vi "Dialog Box.vi"(8 "error in (no error)":errorcluster, 11 "Msg_Error in":refnum<class "Msg_Error.lvclass">) -> (0 "error out":errorcluster, 1 "timed out?":bool, 2 "Selection":string, 3 "Msg_Error out":refnum<class "Msg_Error.lvclass">)   [LabVIEW 2012, in "Msg_Error.lvlib" / "Msg_Error.lvclass"]
doc: "This VI contains the code for the dialog box.\nOverride this VI to provide more functionality or to create your own application-specific dialog box."
uses:
  Msg_Error.lvclass
  Msg_Error.lvclass/Msg_Error.ctl
  <vilib>/Utility/error.llb/DialogType.ctl
  Fading/_Fade In(I32).vi
panel:
  out "String":string
  out "Error Code":string
  in  "Show details":bool
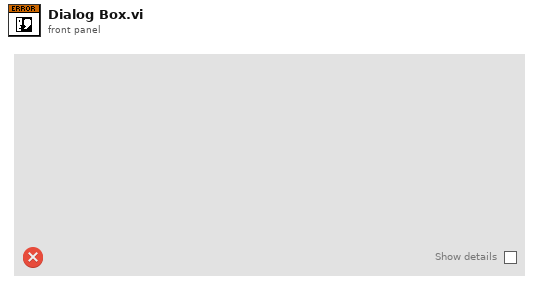
[diagram p1: front panel]
types:
  T1 = typedef "DialogType.ctl" = u16
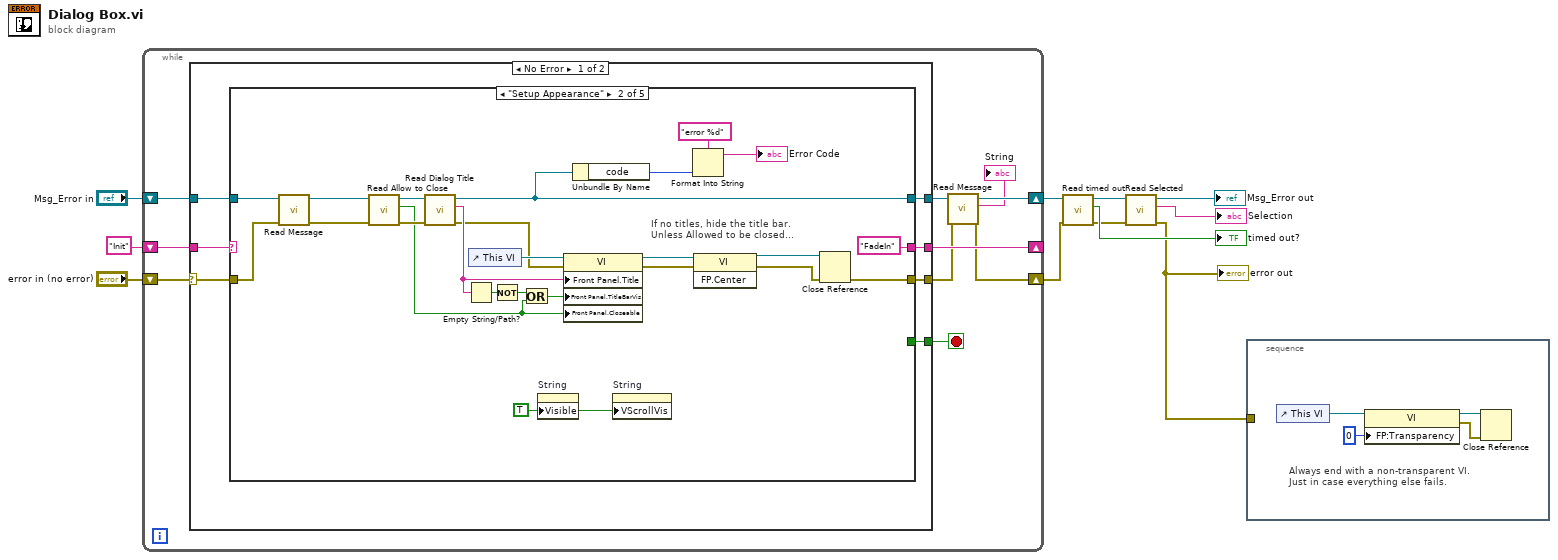
[diagram p0: block diagram]
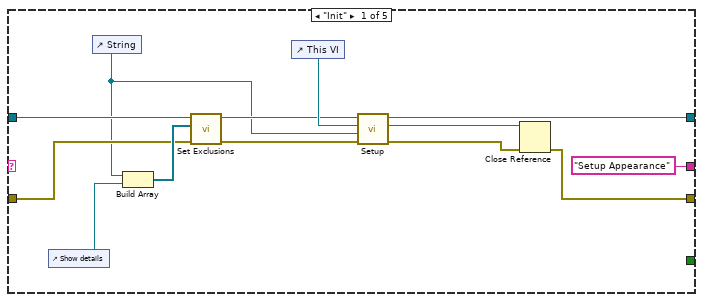
[diagram p2: hidden frame]
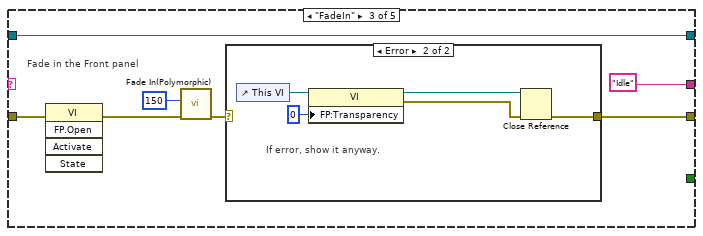
[diagram p3: hidden frame]
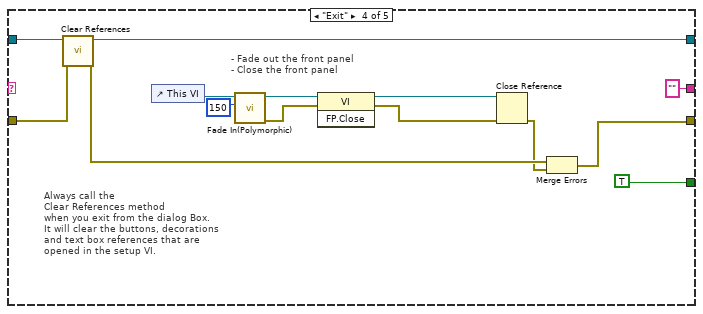
[diagram p5: hidden frame]
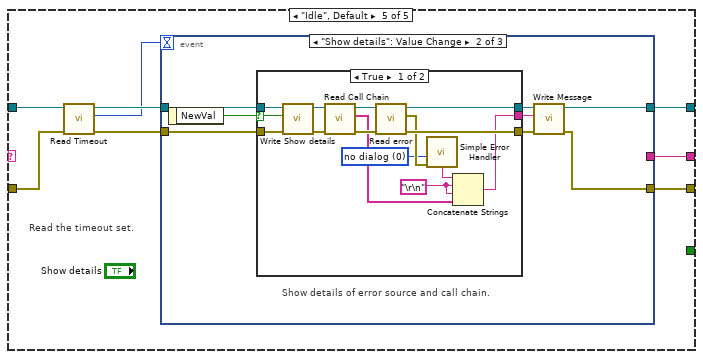
[diagram p6: hidden frame]
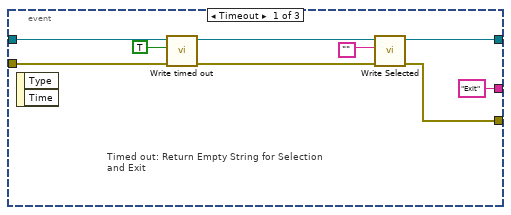
[diagram p7: hidden frame]
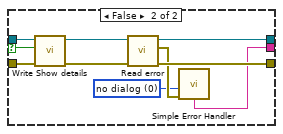
[diagram p8: hidden frame]
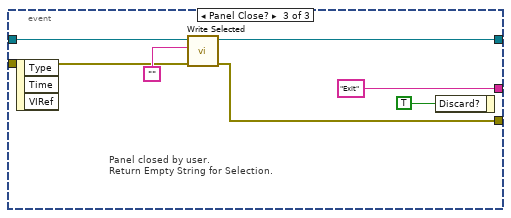
[diagram p9: hidden frame]
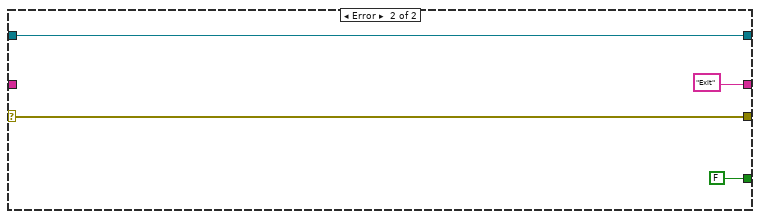
[diagram p10: hidden frame]
diagram:
  n1 = while {
    shift-right: [w19] -> _
    shift-left: "Init" -> [w20]
    shift-right: [w16] -> w5
    shift-left: "Msg_Error in" -> [w21]
    shift-right: [w13] -> w4
    shift-left: "error in (no error)" -> [w17]
    stop <- w18 stop-if-true
    n2 = case shown="No Error" w17 {
      selector: w17 -> [w22 w152]
      tunnel: [w28 w153] -> w15
      tunnel: w21 -> [w27 w153]
      tunnel: [w26 w152] -> w12
      tunnel: w20 -> [w25 _]
      tunnel: [w24 "Exit"] -> w19
      tunnel: [w23 FALSE] -> w18
      frame No Error {
        n3 = case shown="\"Setup Appearance\"" w25 {
          tunnel: [w39 w46 w72 w87 w100] -> w28
          tunnel: w27 -> [w34 w50 w72 w88 w97]
          tunnel: [w40 w57 w68 w86 w99] -> w26
          tunnel: w22 -> [w32 w48 w67 w79 w94]
          tunnel: ["Setup Appearance" "FadeIn" "Idle" "" w98] -> w24
          tunnel: [_ _ _ TRUE _] -> w23
          frame "Init" {
            n4 = control-ref of="Show details"() -> (w29:refnum<vi>)
            n5 = control-ref of="String"() -> (w30:refnum<vi>)
            n6 = Build Array(w30, w29) -> (w35:refnum<vi>[])
            n7 = call-dynamic "Set Exclusions.vi"("error in (no error)"=w32, "Exclusions"=w35, "Dialog in"=w34) -> ("error out"=w31:errorcluster, "Dialog out"=w33:refnum<class "Msg_Error.lvclass">)  [unwired: 7 out]
            n8 = control-ref of="This VI"() -> (w37:refnum<vi>)
            n9 = call-dynamic "Setup.vi"("error in (no error)"=w31, "Str Refnum"=w30, "VI Reference"=w37, "Msg_Error in"=w33) -> ("error out"=w36:errorcluster, "VI reference (dup)"=w38:refnum<vi>, "Msg_Error out"=w39:refnum<class "Msg_Error.lvclass">)  [unwired: 5 out]
            n10 = Close Reference(reference=w38, error in (no error)=w36) -> (error out=w40:errorcluster)
          }
          frame "Setup Appearance" {
            w42 = TRUE ("Visible")
            # "If no titles, hide the title bar.\nUnless Allowed to be closed..."
            n11 = call-dynamic "Read Message.vi"("error in (no error)"=w48, "Dialog in"=w50) -> ("error out"=w47:errorcluster, "Dialog out"=w49:refnum<class "Msg_Error.lvclass">)  [unwired: 7 in, 1 out]
            n12 = call-dynamic "Read Allow to Close.vi"("error in (no error)"=w47, "Dialog.lvclass in"=w49) -> ("error out"=w54:errorcluster, "Allow to close?"=w51:bool, "Dialog.lvclass out"=w55:refnum<class "Msg_Error.lvclass">)  [unwired: 7 out]
            n13 = call-dynamic "Read Dialog Title.vi"("error in (no error)"=w54, "Dialog in"=w55) -> ("error out"=w56:errorcluster, "Dialog Title"=w60:string, "Dialog out"=w46:refnum<class "Msg_Error.lvclass">)  [unwired: 7 out]
            n14 = Empty String/Path?(string/path=w60) -> (empty?=w63:bool)
            n15 = control-ref of="This VI"() -> (w64:refnum<vi>)
            n16 = Not(x=w63) -> (.not. x?=w53:bool)
            n17 = Or(x=w53, y=w51) -> (x .or. y?=w52:bool)
            n18 = property on="String" class="Str"("Visible"=w42) -> ()  [unwired: 2 in, 2 out]
            n19 = property class="VI"(reference=w64, error in=w56, "Front Panel.Title"=w60, "Front Panel.TitleBarVis"=w52, "Front Panel.Closeable"=w51) -> (reference out=w62:refnum<vi>, error out=w61:errorcluster)
            n20 = Unbundle By Name(w46) -> ("code"=w45:i32)
            n21 = property on="String" class="Str"("VScrollVis"=w42) -> ()  [unwired: 2 in, 2 out]
            n22 = Format Into String(format string="error %d", w45) -> (resulting string=→"Error Code":string)  [unwired: 2 in, 1 out]
            n23 = invoke class="VI" method="FP.Center"(reference=w62, error in=w61) -> (reference out=w59:refnum<vi>, error out=w58:errorcluster)  [unwired: 1 in, 1 out]
            n24 = Close Reference(reference=w59, error in (no error)=w58) -> (error out=w57:errorcluster)
          }
          frame "FadeIn" {
            # "Fade in the Front panel"
            n25 = invoke class="VI" method="FP.Open"(error in=w67) -> (error out=w66:errorcluster)  [unwired: 4 in, 4 out]
            n26 = call-poly "Fade In(Polymorphic).vi"("error in"=w66, "Fade time (ms)"=150) -> ("error out"=w69:errorcluster)  [unwired: 2 in, 7 out]
            n27 = case shown="Error" w69 {
              selector: w69 -> [w73 _]
              tunnel: [w73 w74] -> w68
              frame No Error {
              }
              frame Error {
                # "If error, show it anyway."
                n28 = control-ref of="This VI"() -> (w76:refnum<vi>)
                n29 = property class="VI"(reference=w76, "FP:Transparency"=u8 0 ("Front Panel Window:Transparency")) -> (reference out=w77:refnum<vi>, error out=w78:errorcluster)  [unwired: 1 in]
                n30 = Close Reference(reference=w77, error in (no error)=w78) -> (error out=w74:errorcluster)
              }
            }
          }
          frame "Exit" {
            # "Always call the\nClear References method\nwhen you exit from the dialog Box.\nIt will clear the buttons, decorations\nand text box references that are \nopened in the setup VI."
            # "- Fade out the front panel\n- Close the front panel"
            n31 = call-dynamic "Clear References.vi"("error in (no error)"=w79, "Dialog in"=w88) -> ("error out"=w81:errorcluster, "Dialog out"=w87:refnum<class "Msg_Error.lvclass">)  [unwired: 8 out]
            n32 = control-ref of="This VI"() -> (w89:refnum<vi>)
            n33 = call-poly "Fade In(Polymorphic).vi"("Fade time (ms)"=150, "VI Reference (calling VI)"=w89) -> ("error out"=w85:errorcluster, "dup VI Reference"=w84:refnum<vi>)  [unwired: 2 in, 6 out]
            n34 = invoke class="VI" method="FP.Close"(reference=w84, error in=w85) -> (reference out=w82:refnum<vi>, error out=w83:errorcluster)  [unwired: 1 in, 1 out]
            n35 = Close Reference(reference=w82, error in (no error)=w83) -> (error out=w80:errorcluster)
            n36 = Merge Errors(w81, w80) -> (w86:errorcluster)
          }
          frame "Idle", Default {
            # "Read the timeout set."
            n37 = call-dynamic "Read Timeout.vi"("error in (no error)"=w94, "Dialog.lvclass in"=w97) -> ("error out"=w93:errorcluster, "Timeout"=w95:i32, "Dialog.lvclass out"=w96:refnum<class "Msg_Error.lvclass">)  [unwired: 7 out]
            n38 = event shown="[1] \"Show details\": Value Change" {
              selector: _ -> [_ _ _]
              dyn-events: _ -> [_ _ _]
              timeout: w95 -> [_ _ _]
              tunnel: [w102 w115 w145] -> w100
              tunnel: w96 -> [w108 w112 w146]
              tunnel: [w103 w116 w143] -> w99
              tunnel: w93 -> [w106 w111 w144]
              tunnel: ["Exit" _ "Exit"] -> w98
              event Timeout {
                # "Timed out: Return Empty String for Selection\nand Exit"
                n39 = event-data() -> ()  [unwired: 3 out]
                n40 = call-dynamic "Write timed out.vi"("error in (no error)"=w106, "timed out?"=TRUE, "Dialog.lvclass in"=w108) -> ("error out"=w104:errorcluster, "Dialog.lvclass out"=w105:refnum<class "Msg_Error.lvclass">)  [unwired: 7 out]
                n41 = call-dynamic "Write Selected.vi"("error in (no error)"=w104, "Selected"="", "Dialog.lvclass in"=w105) -> ("error out"=w103:errorcluster, "Dialog.lvclass out"=w102:refnum<class "Msg_Error.lvclass">)  [unwired: 7 out]
              }
              event "Show details": Value Change {
                # "Show details of error source and call chain."
                n42 = event-data() -> ("NewVal"=w110:bool)  [unwired: 1 out]
                n43 = case shown="True" w110 {
                  selector: w110 -> [w118 w136]
                  tunnel: [w130 w142] -> w117
                  tunnel: [w129 w133] -> w114
                  tunnel: [w128 w141] -> w113
                  tunnel: w112 -> [w120 w138]
                  tunnel: w111 -> [w119 w137]
                  frame True {
                    w122 = "\r\n"
                    w121 = T1 0 items=["no dialog", "OK message", "continue or stop message", "OK message + warnings", "continue/stop + warnings"] ("type of dialog (OK msg:1)")
                    n44 = call-dynamic "Write Show details.vi"("error in (no error)"=w119, "Show details"=w118, "Msg_Error.lvclass in"=w120) -> ("error out"=w132:errorcluster, "Msg_Error.lvclass out"=w131:refnum<class "Msg_Error.lvclass">)  [unwired: 7 out]
                    n45 = call-dynamic "Read Call Chain.vi"("error in (no error)"=w132, "Msg_Error.lvclass in"=w131) -> ("error out"=w127:errorcluster, "Call Chain"=w126:string[], "Msg_Error.lvclass out"=w125:refnum<class "Msg_Error.lvclass">)  [unwired: 7 out]
                    n46 = call-dynamic "Read error.vi"("error in (no error)"=w127, "Msg_Error.lvclass in"=w125) -> ("error out"=w130:errorcluster, "error"=w124:errorcluster, "Msg_Error.lvclass out"=w128:refnum<class "Msg_Error.lvclass">)  [unwired: 7 out]
                    n47 = call <vilib>:"Simple Error Handler.vi"("type of dialog (OK msg:1)"=w121, "error in (no error)"=w124) -> ("message"=w123:string)  [unwired: 1 in, 6 out]
                    n48 = Concatenate Strings(w123, w122, w122, w126) -> (w129:string)
                  }
                  frame False {
                    w139 = T1 0 items=["no dialog", "OK message", "continue or stop message", "OK message + warnings", "continue/stop + warnings"] ("type of dialog (OK msg:1)")
                    n49 = call-dynamic "Write Show details.vi"("error in (no error)"=w137, "Show details"=w136, "Msg_Error.lvclass in"=w138) -> ("error out"=w134:errorcluster, "Msg_Error.lvclass out"=w135:refnum<class "Msg_Error.lvclass">)  [unwired: 7 out]
                    n50 = call-dynamic "Read error.vi"("error in (no error)"=w134, "Msg_Error.lvclass in"=w135) -> ("error out"=w142:errorcluster, "error"=w140:errorcluster, "Msg_Error.lvclass out"=w141:refnum<class "Msg_Error.lvclass">)  [unwired: 7 out]
                    n51 = call <vilib>:"Simple Error Handler.vi"("type of dialog (OK msg:1)"=w139, "error in (no error)"=w140) -> ("message"=w133:string)  [unwired: 1 in, 6 out]
                  }
                }
                n52 = call-dynamic "Write Message.vi"("error in (no error)"=w117, "Message"=w114, "Dialog in"=w113) -> ("error out"=w116:errorcluster, "Dialog out"=w115:refnum<class "Msg_Error.lvclass">)  [unwired: 7 out]
              }
              event Panel Close? {
                # "Panel closed by user.\nReturn Empty String for Selection."
                n53 = event-data() -> ()  [unwired: 4 out]
                n54 = call-dynamic "Write Selected.vi"("error in (no error)"=w144, "Selected"="", "Dialog.lvclass in"=w146) -> ("error out"=w143:errorcluster, "Dialog.lvclass out"=w145:refnum<class "Msg_Error.lvclass">)  [unwired: 7 out]
                n55 = event-data("Discard?"=TRUE) -> ()  [unwired: 1 in, 1 out]
              }
            }
          }
        }
      }
      frame Error {
      }
    }
    n56 = call-dynamic "Read Message.vi"("error in (no error)"=w12, "Dialog in"=w15) -> ("error out"=w13:errorcluster, "Message"=→"String":string, "Dialog out"=w16:refnum<class "Msg_Error.lvclass">)  [unwired: 7 in]
  }
  n57 = call-dynamic "Read timed out.vi"("error in (no error)"=w4, "Dialog.lvclass in"=w5) -> ("error out"=w2:errorcluster, "timed out?"=→"timed out?":bool, "Dialog.lvclass out"=w3:refnum<class "Msg_Error.lvclass">)  [unwired: 7 out]
  n58 = call-dynamic "Read Selected.vi"("error in (no error)"=w2, "Dialog.lvclass in"=w3) -> ("error out"=w1:errorcluster, "Selected"=→"Selection":string, "Dialog.lvclass out"=→"Msg_Error out":refnum<class "Msg_Error.lvclass">)  [unwired: 7 out]
  "error out" <- w1
  n59 = stacked-sequence {
    tunnel: w1 -> [_]
    frame #0 {
      # "Always end with a non-transparent VI.\nJust in case everything else fails."
      n60 = control-ref of="This VI"() -> (w156:refnum<vi>)
      n61 = property class="VI"(reference=w156, "FP:Transparency"=u8 0 ("Front Panel Window:Transparency")) -> (reference out=w155:refnum<vi>, error out=w154:errorcluster)  [unwired: 1 in]
      n62 = Close Reference(reference=w155, error in (no error)=w154) -> ()  [unwired: 1 out]
    }
  }
